vi "Operating Voltage.vi"(8 "error in (no error)":errorcluster) -> (0 "error out":errorcluster)   [LabVIEW 2025]
uses:
  SubVIs/All test cluster.ctl
  SubVIs/All_enum_ctl.ctl
  SubVIs/Arduino_lamps.ctl
  SubVIs/Lamps_global.vi
  <vilib>/Utility/file.llb/Write Delimited Spreadsheet (string).vi
  <instrlib>/BK Precision 9200 Series/BK Precision 9200 Series.lvlib
  <instrlib>/Keithley 2260B/Keithley 2260B.lvlib
panel:
  in  "ESP COM PORT":refnum<visa-resource-name>
  out "Connected? 2":bool caption="Long Blank Button"
  out "Status":string
  in  "POWER SUPPLY":bool caption="Blank Button"
  out "Text name":string
  in  "PS COM PORT":refnum<visa-resource-name>
  in  "Start/Stop":bool caption="Slide Switch"
  in  "File Path:":path
  in  "FILENAME":string
  out "Table":string[][](table)
  out "Connected?":bool caption="Long Blank Button"
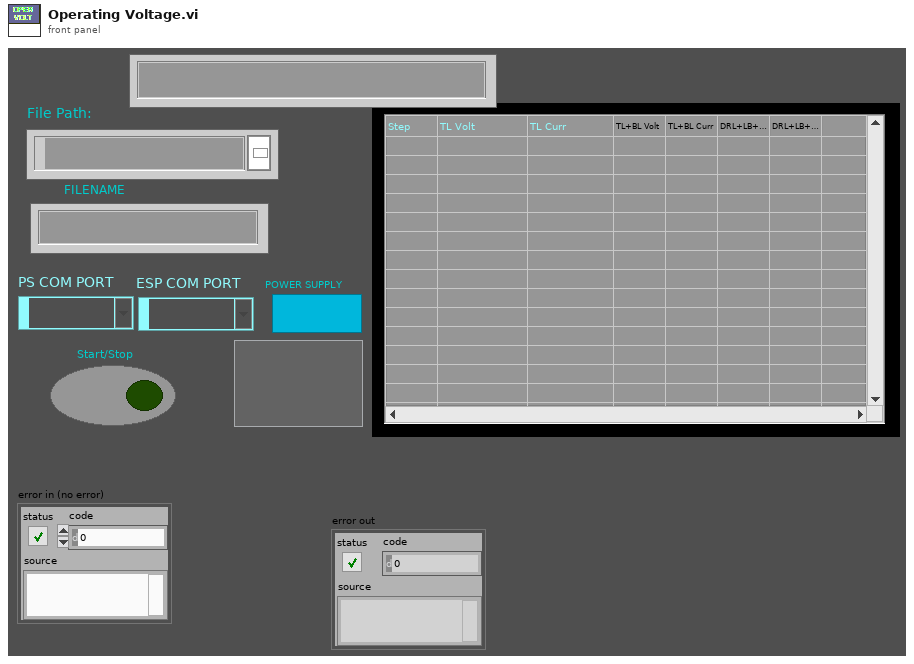
[diagram p1: front panel]
types:
  T1 = enum32{"Invalid", "Standard", "Closed", "Hidden", "Minimized", "Maximized"}
  T2 = typedef "All_enum_ctl.ctl" = enum16{"Init", "Poll", "Connect_esp32", "Connect", "check_start", "Start", "Set_Voltage", "On_relay", "Read_Voltage", "Off_Relay", "Next_Relay", "Next_Step", "Stop", "Store", "Error", "Exit"}
  T3 = typedef "All test cluster.ctl" = cluster{"FilePath":path, "Test Status":bool, "Start Volt":dbl, "End Volt":dbl, "Present Step":dbl, "Present Time(s)":dbl, "End Time":dbl, "Table":string[], "Intensity":string, "BK/Keith":bool, "COM":refnum<visa-resource-name>, "Next state":T2, "Step no.":dbl, "Start ms":u32, "ESP_COM":refnum<visa-resource-name>, "Relay_no":dbl, "Datas":string[]}
  T4 = typedef "Arduino_lamps.ctl" = enum16{"Init", "Poll", "Read", "Write", "Exit"}
  T5 = cluster{"Baud Rate":u32, "Parity":u16, "Data Bits":u16, "Stop Bits":u16, "Flow Control":u16}
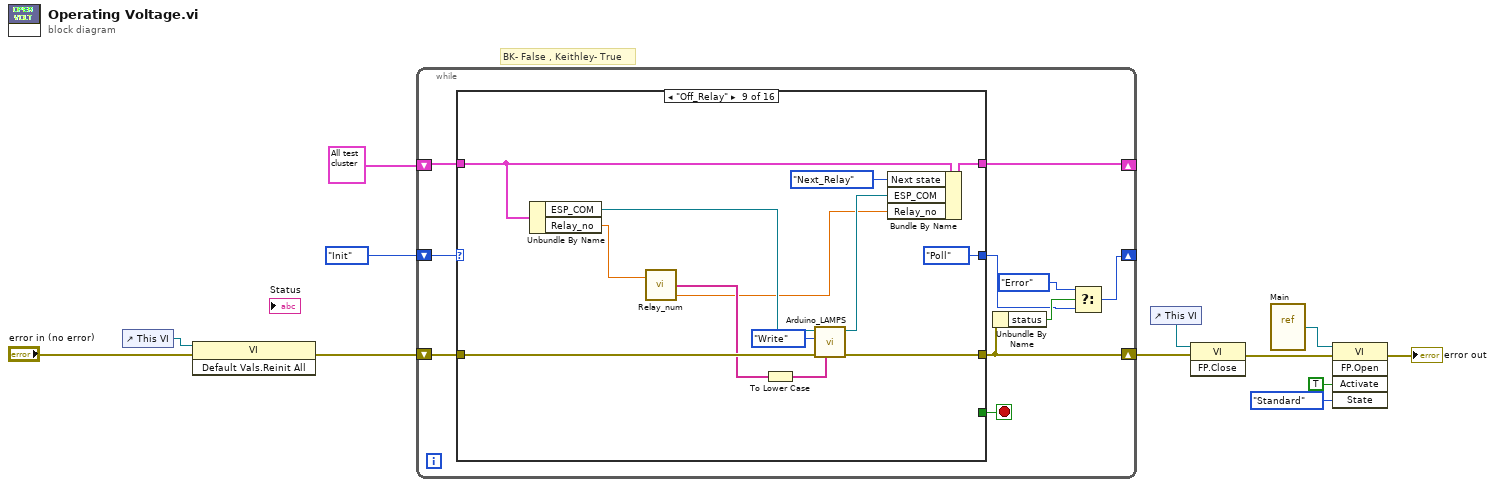
[diagram p0: block diagram]
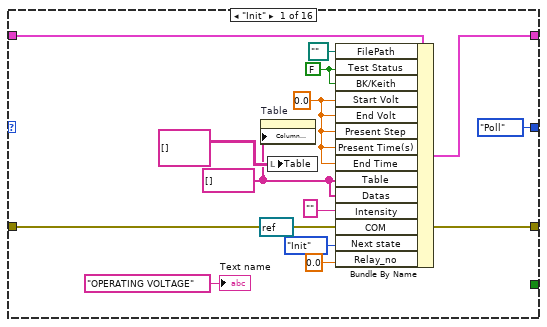
[diagram p2: hidden frame]
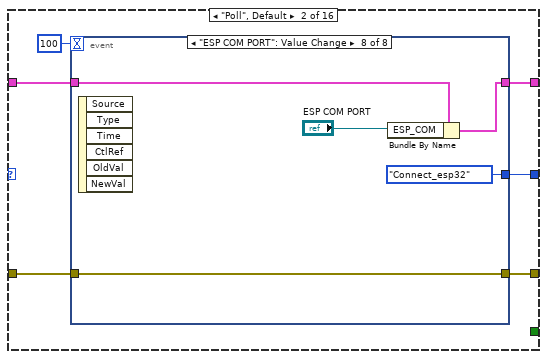
[diagram p3: hidden frame]
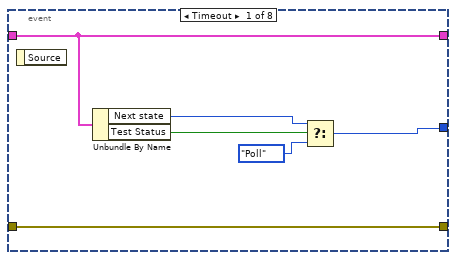
[diagram p4: hidden frame]
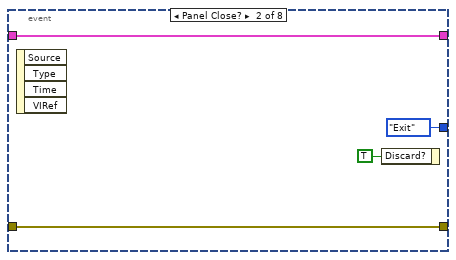
[diagram p5: hidden frame]
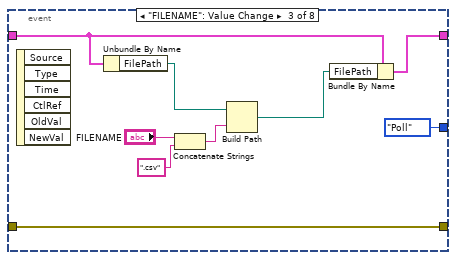
[diagram p6: hidden frame]
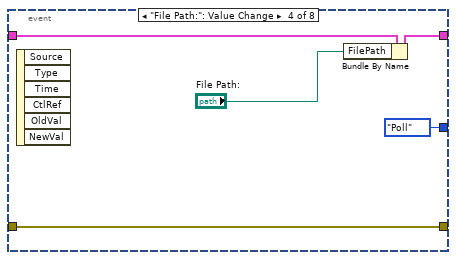
[diagram p7: hidden frame]
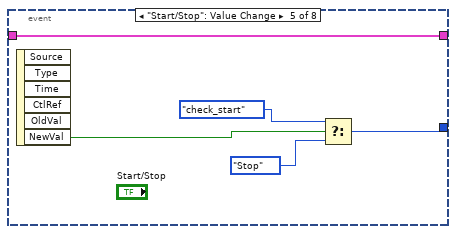
[diagram p8: hidden frame]
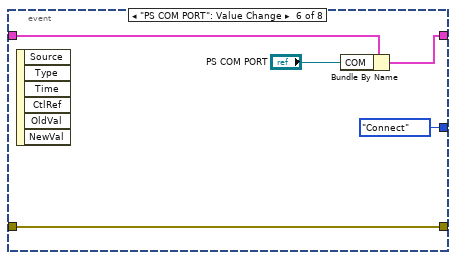
[diagram p9: hidden frame]
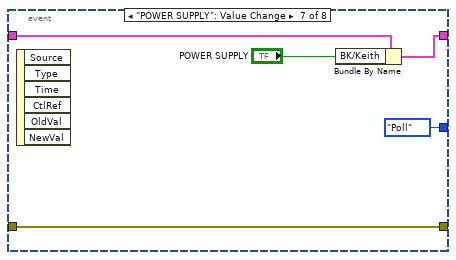
[diagram p10: hidden frame]
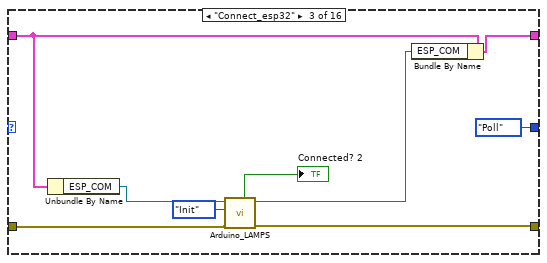
[diagram p11: hidden frame]
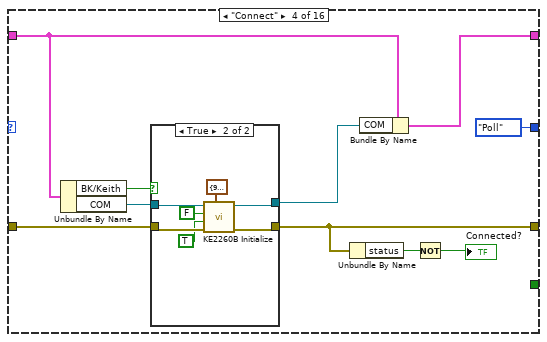
[diagram p12: hidden frame]
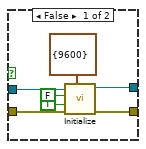
[diagram p13: hidden frame]
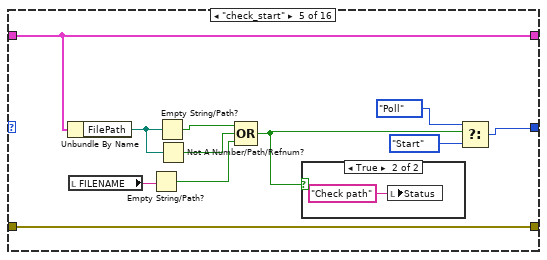
[diagram p14: hidden frame]
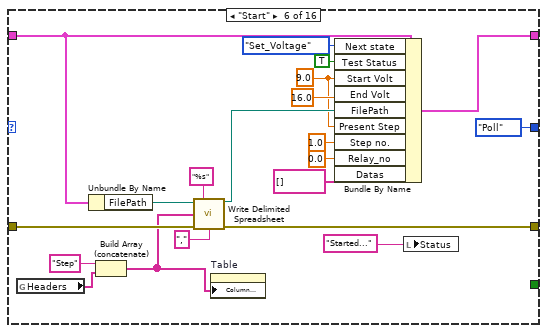
[diagram p16: hidden frame]
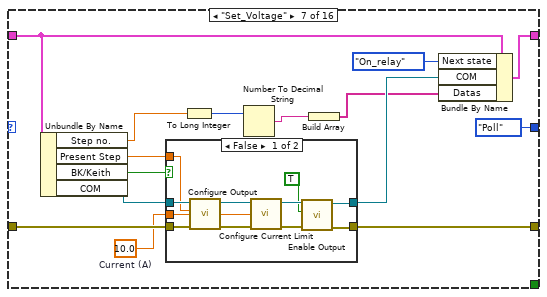
[diagram p17: hidden frame]
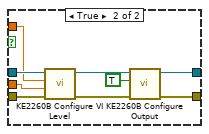
[diagram p18: hidden frame]
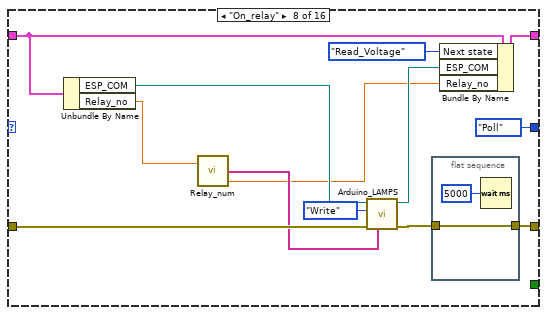
[diagram p19: hidden frame]
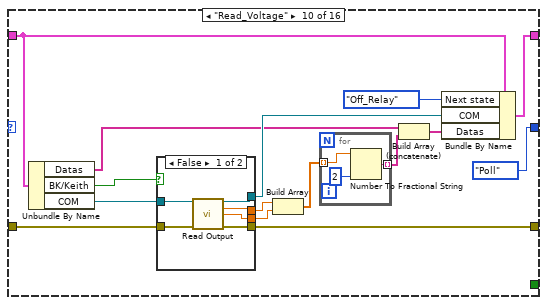
[diagram p20: hidden frame]
diagram:
  # "BK- False , Keithley- True"
  n1 = control-ref of="This VI"() -> (w12:refnum<vi>)
  n2 = invoke class="VI" method="Default Vals.Reinit All"(reference=w12, error in="error in (no error)") -> (error out=w10:errorcluster)  [unwired: 1 in, 2 out]
  n3 = while {
    shift-right: [w21] -> _
    shift-left: T3 {"FilePath"=path "", "Test Status"=FALSE, "Start Volt"=0.0, "End Volt"=0.0, "Present Step"=0.0, "Present Time(s)"=0.0, "End Time"=0.0, "Table"=[], "Intensity"="", "BK/Keith"=FALSE, "COM"="", "Next state"=enum."Init", "Step no."=0.0, "Start ms"=0, "ESP_COM"="", "Relay_no"=0.0, "Datas"=[]} -> [w20]
    shift-right: [w17] -> w2
    shift-left: w10 -> [w19]
    shift-right: [w13] -> _
    shift-left: All_enum_ctl."Init" -> [w22]
    stop <- w18 stop-if-true
    n4 = case shown="\"Off_Relay\"" w22 {
      tunnel: [w34 w39 w94 w97 w129 w150 w165 w194 w209 w224 w255 w265 w292 w306 w324 w344] -> w21
      tunnel: w20 -> [w36 w40 w93 w101 w129 w144 w164 w198 w213 w228 w258 w264 w290 w307 w327 w344]
      tunnel: w19 -> [w35 w42 w92 w105 w130 w146 w166 w199 w214 w229 w259 w267 w288 w311 w331 w349]
      tunnel: [w35 w41 w91 w100 w130 w145 w156 w190 w203 w227 w252 w267 w287 w311 w329 w345] -> w17
      tunnel: [All_enum_ctl."Poll" w37 All_enum_ctl."Poll" All_enum_ctl."Poll" w121 All_enum_ctl."Poll" All_enum_ctl."Poll" All_enum_ctl."Poll" All_enum_ctl."Poll" All_enum_ctl."Poll" All_enum_ctl."Poll" All_enum_ctl."Poll" All_enum_ctl."Poll" All_enum_ctl."Poll" All_enum_ctl."Poll" All_enum_ctl."Exit"] -> w14
      tunnel: [_ _ _ _ _ _ _ _ _ _ _ _ _ _ _ TRUE] -> w18
      frame "Init" {
        w23 = string[] [] ("Table")
        w32 = 0.0 ("Start Volt")
        w30 = FALSE ("Test Status")
        n5 = property on="Table" class="Tbl (strict)"("Column Headers[]"=w23) -> ()  [unwired: 2 in, 2 out]
        n6 = local write "Table"(string[][] [] ("Table")) -> ()
        n7 = Bundle By Name(cluster=w36, "FilePath"=path "", "Test Status"=w30, "BK/Keith"=w30, "Start Volt"=w32, "End Volt"=w32, "Present Step"=w32, "Present Time(s)"=w32, "End Time"=w32, "Table"=w23, "Datas"=w23, "Intensity"="", "COM"=refnum<visa-resource-name> refnum, "Next state"=All_enum_ctl."Init" ("Last state"), "Relay_no"=0.0) -> (w34:T3)
        "Text name" <- "OPERATING VOLTAGE" ("Text name")
      }
      frame "Poll", Default {
        n8 = event shown="[7] \"ESP COM PORT\": Value Change" {
          selector: _ -> [_ _ _ _ _ _ _ _]
          dyn-events: _ -> [_ _ _ _ _ _ _ _]
          timeout: 100 -> [_ _ _ _ _ _ _ _]
          tunnel: w42 -> [w48 w49 w61 w64 _ w72 w77 w82]
          tunnel: [w48 w49 w61 w64 _ w72 w77 w82] -> w41
          tunnel: w40 -> [w47 w50 w59 w66 w70 w76 w81 w85]
          tunnel: [w47 w50 w55 w63 w70 w75 w80 w86] -> w39
          tunnel: [w43 All_enum_ctl."Exit" ("f") All_enum_ctl."Poll" All_enum_ctl."Poll" w67 All_enum_ctl."Connect" ("f") All_enum_ctl."Poll" ("f") All_enum_ctl."Connect_esp32" ("f")] -> w37
          event Timeout {
            n9 = event-data() -> ()  [unwired: 1 in, 1 out]
            n10 = Unbundle By Name(w47) -> ("Next state"=w44:T2, "Test Status"=w46:bool)
            n11 = Select(t=w44, s=w46, f=All_enum_ctl."Poll") -> (s? t:f=w43:T2)
          }
          event Panel Close? {
            n12 = event-data() -> ()  [unwired: 1 in, 4 out]
            n13 = event-data("Discard?"=TRUE) -> ()  [unwired: 1 in, 1 out]
          }
          event "FILENAME": Value Change {
            n14 = event-data() -> ()  [unwired: 1 in, 6 out]
            n15 = Unbundle By Name(w59) -> ("FilePath"=w58:path)
            n16 = Concatenate Strings("FILENAME", ".csv" ("string")) -> (w57:string)
            n17 = Build Path(base path=w58, name or relative path=w57) -> (appended path=w54:path)
            n18 = Bundle By Name(cluster=w59, "FilePath"=w54) -> (w55:T3)
          }
          event "File Path:": Value Change {
            n19 = event-data() -> ()  [unwired: 1 in, 6 out]
            n20 = Bundle By Name(cluster=w66, "FilePath"="File Path:") -> (w63:T3)
          }
          event "Start/Stop": Value Change {
            n21 = event-data() -> ("NewVal"=w71:bool)  [unwired: 1 in, 5 out]
            n22 = Select(t=All_enum_ctl."check_start", s=w71, f=All_enum_ctl."Stop") -> (s? t:f=w67:T2)
          }
          event "PS COM PORT": Value Change {
            n23 = event-data() -> ()  [unwired: 1 in, 6 out]
            n24 = Bundle By Name(cluster=w76, "COM"="PS COM PORT") -> (w75:T3)
          }
          event "POWER SUPPLY": Value Change {
            n25 = event-data() -> ()  [unwired: 1 in, 6 out]
            n26 = Bundle By Name(cluster=w81, "BK/Keith"="POWER SUPPLY") -> (w80:T3)
          }
          event "ESP COM PORT": Value Change {
            n27 = event-data() -> ()  [unwired: 1 in, 6 out]
            n28 = Bundle By Name(cluster=w85, "ESP_COM"="ESP COM PORT") -> (w86:T3)
          }
        }
      }
      frame "Connect_esp32" {
        n29 = Unbundle By Name(w93) -> ("ESP_COM"=w89:refnum<visa-resource-name>)
        n30 = call "Arduino_LAMPS.vi"("error out"=w92, "Enum"=Arduino_lamps."Init", "VISA resource name"=w89) -> ("error out 2"=w91:errorcluster, "VISA out"=w88:refnum<visa-resource-name>, "status"=→"Connected? 2":bool)  [unwired: 4 in, 2 out]
        n31 = Bundle By Name(cluster=w93, "ESP_COM"=w88) -> (w94:T3)
      }
      frame "Connect" {
        n32 = Unbundle By Name(w101) -> ("BK/Keith"=w99:bool, "COM"=w98:refnum<visa-resource-name>)
        n33 = case shown="True" w99 {
          tunnel: w105 -> [w112 w119]
          tunnel: [w111 w118] -> w100
          tunnel: w98 -> [w110 w117]
          tunnel: [w106 w115] -> w96
          frame False {
            n34 = call <instrlib>:"Initialize.vi"("Serial Configuration"=cluster{"Baud Rate":u32} {"Baud Rate"=9600}, "error in (no error)"=w112, "Reset (True)"=TRUE, "ID Query (True)"=FALSE, "VISA resource name"=w110) -> ("error out"=w111:errorcluster, "VISA resource name out"=w106:refnum<visa-resource-name>)  [unwired: 5 in]
          }
          frame True {
            n35 = call <instrlib>:"KE2260B Initialize.vi"("Serial Configuration"=T5 {"Baud Rate"=9600, "Parity"=0, "Data Bits"=8, "Stop Bits"=10, "Flow Control"=0}, "error in (no error)"=w119, "Reset (True)"=TRUE, "ID Query (True)"=FALSE, "VISA resource name"=w117) -> ("error out"=w118:errorcluster, "VISA resource name out"=w115:refnum<visa-resource-name>)  [unwired: 5 in]
          }
        }
        n36 = Unbundle By Name(w100) -> ("status"=w104:bool)
        n37 = Bundle By Name(cluster=w101, "COM"=w96) -> (w97:T3)
        n38 = Not(x=w104) -> (.not. x?=→"Connected?":bool)
      }
      frame "check_start" {
        n39 = Unbundle By Name(w129) -> ("FilePath"=w127:path)
        n40 = local read "FILENAME"() -> (w128:string)
        n41 = Empty String/Path?(string/path=w128) -> (empty?=w124:bool)
        n42 = Empty String/Path?(string/path=w127) -> (empty?=w126:bool)
        n43 = Not A Number/Path/Refnum?(number/path/refnum=w127) -> (NaN/Path/Refnum?=w125:bool)
        n44 = Compound Arithmetic op=OR(w126, w125, w124) -> (w120:bool)
        n45 = case shown="True" w120 {
          frame False {
          }
          frame True {
            n46 = local write "Status"("Check path") -> ()
          }
        }
        n47 = Select(t=All_enum_ctl."Poll", s=w120, f=All_enum_ctl."Start") -> (s? t:f=w121:T2)
      }
      frame "Start" {
        w139 = 9.0 ("Start Volt")
        n48 = global read "Lamps_global.vi" "Headers"() -> (w133:string[])
        n49 = Unbundle By Name(w144) -> ("FilePath"=w143:path)
        n50 = Build Array (concatenate)("Step" ("String"), w133) -> (w132:string[])
        n51 = call-poly <vilib>:"Write Delimited Spreadsheet.vi"("file path (dialog if empty)"=w143, "format (%s)"="%s" ("format (%.3f)"), "1D data"=w132, "error in (no error)"=w146, "delimiter (\\t)"="," ("delimiter (\\t)")) -> ("new file path (Not A Path if cancelled)"=w140:path, "error out"=w145:errorcluster)  [unwired: 9 in]
        n52 = property on="Table" class="Tbl (strict)"("Column Headers[]"=w132) -> ()  [unwired: 2 in, 2 out]
        n53 = Bundle By Name(cluster=w144, "Next state"=All_enum_ctl."Set_Voltage" ("Last state"), "Test Status"=TRUE, "Start Volt"=w139, "End Volt"=16.0, "FilePath"=w140, "Present Step"=w139, "Step no."=1.0, "Relay_no"=0.0, "Datas"=string[] []) -> (w150:T3)
        n54 = local write "Status"("Started...") -> ()
      }
      frame "Set_Voltage" {
        w158 = 10.0  # Current (A)
        n55 = Unbundle By Name(w164) -> ("Step no."=w155:dbl, "Present Step"=w159:dbl, "BK/Keith"=w160:bool, "COM"=w163:refnum<visa-resource-name>)
        n56 = case shown="False" w160 {
          tunnel: w166 -> [w170 w186]
          tunnel: [w177 w185] -> w156
          tunnel: w163 -> [w175 w183]
          tunnel: [w176 w181] -> w162
          tunnel: w159 -> [w174 w179]
          tunnel: w158 -> [w168 w178]
          frame False {
            n57 = call <instrlib>:"Configure Output.vi"("error in (no error)"=w170, "Voltage Level (0.0 V)"=w174, "VISA resource name"=w175) -> ("error out"=w171:errorcluster, "VISA resource name out"=w169:refnum<visa-resource-name>)  [unwired: 7 in]
            n58 = call <instrlib>:"Configure Current Limit.vi"("error in (no error)"=w171, "Current Limit (0.0 A)"=w168, "VISA resource name"=w169) -> ("error out"=w173:errorcluster, "VISA resource name out"=w172:refnum<visa-resource-name>)  [unwired: 7 in]
            n59 = call <instrlib>:"Enable Output.vi"("error in (no error)"=w173, "Enable Output (F: False)"=TRUE, "VISA resource name"=w172) -> ("error out"=w177:errorcluster, "VISA resource name out"=w176:refnum<visa-resource-name>)  [unwired: 7 in]
          }
          frame True {
            n60 = call <instrlib>:"KE2260B Configure VI Level.vi"("error in (no error)"=w186, "Current Level (0.000 A)"=w178, "Voltage Level (0.000 V)"=w179, "VISA resource name"=w183) -> ("error out"=w184:errorcluster, "VISA resource name out"=w182:refnum<visa-resource-name>)  [unwired: 6 in]
            n61 = call <instrlib>:"KE2260B Configure Output.vi"("error in (no error)"=w184, "Enable Output (T: Enable)"=TRUE, "VISA resource name"=w182) -> ("error out"=w185:errorcluster, "VISA resource name out"=w181:refnum<visa-resource-name>)  [unwired: 7 in]
          }
        }
        n62 = To Long Integer(number=w155) -> (32bit integer=w154:i32)
        n63 = Number To Decimal String(number=w154) -> (decimal integer string=w153:string)  [unwired: 1 in]
        n64 = Build Array(w153) -> (w152:string[])
        n65 = Bundle By Name(cluster=w164, "Next state"=All_enum_ctl."On_relay", "COM"=w162, "Datas"=w152) -> (w165:T3)
      }
      frame "On_relay" {
        n66 = Unbundle By Name(w198) -> ("ESP_COM"=w197:refnum<visa-resource-name>, "Relay_no"=w189:dbl)
        n67 = call "Relay_num.vi"("Relay_no."=w189) -> ("Relay"=w188:string[], "Relay_no.out"=w187:dbl)  [unwired: 1 in, 1 out]
        n68 = call "Arduino_LAMPS.vi"("DO's"=w188, "error out"=w199, "Enum"=Arduino_lamps."Write", "VISA resource name"=w197) -> ("error out 2"=w191:errorcluster, "VISA out"=w193:refnum<visa-resource-name>)  [unwired: 3 in, 3 out]
        n69 = flat-sequence {
          tunnel: w191 -> [w201]
          tunnel: [w201] -> w190
          frame #0 {
            n70 = Wait (ms)(milliseconds to wait=u32 5000) -> ()  [unwired: 1 out]
          }
        }
        n71 = Bundle By Name(cluster=w198, "Next state"=All_enum_ctl."Read_Voltage", "ESP_COM"=w193, "Relay_no"=w187) -> (w194:T3)
      }
      frame "Off_Relay" {
        n72 = Unbundle By Name(w213) -> ("ESP_COM"=w212:refnum<visa-resource-name>, "Relay_no"=w206:dbl)
        n73 = call "Relay_num.vi"("Relay_no."=w206) -> ("Relay"=w205:string[], "Relay_no.out"=w204:dbl)  [unwired: 1 in, 1 out]
        n74 = To Lower Case(string=w205) -> (all lower case string=w202:string[])
        n75 = call "Arduino_LAMPS.vi"("DO's"=w202, "error out"=w214, "Enum"=Arduino_lamps."Write", "VISA resource name"=w212) -> ("error out 2"=w203:errorcluster, "VISA out"=w208:refnum<visa-resource-name>)  [unwired: 3 in, 3 out]
        n76 = Bundle By Name(cluster=w213, "Next state"=All_enum_ctl."Next_Relay", "ESP_COM"=w208, "Relay_no"=w204) -> (w209:T3)
      }
      frame "Read_Voltage" {
        n77 = Unbundle By Name(w228) -> ("Datas"=w216:string[], "BK/Keith"=w225:bool, "COM"=w226:refnum<visa-resource-name>)
        n78 = case shown="False" w225 {
          tunnel: w229 -> [w238 w244]
          tunnel: [w237 w243] -> w227
          tunnel: w226 -> [w236 w241]
          tunnel: [w235 w242] -> w223
          tunnel: [w234 w240] -> w220
          tunnel: [w233 w239] -> w219
          frame False {
            n79 = call <instrlib>:"Read Output.vi"("VISA resource name"=w236, "error in (no error)"=w238) -> ("VISA resource name out"=w235:refnum<visa-resource-name>, "Actual Voltage Level (V)"=w234:dbl, "Actual Current Level (A)"=w233:dbl, "error out"=w237:errorcluster)  [unwired: 9 in, 1 out]
          }
          frame True {
            n80 = call <instrlib>:"KE2260B Read Output.vi"("error in (no error)"=w244, "VISA resource name"=w241) -> ("error out"=w243:errorcluster, "Actual Current Level (A)"=w239:dbl, "Actual Voltage Level (V)"=w240:dbl, "VISA resource name out"=w242:refnum<visa-resource-name>)  [unwired: 6 in]
          }
        }
        n81 = Build Array(w220, w219) -> (w218:dbl[])
        n82 = for {
          tunnel: w218 -> [w231] mode=indexing
          tunnel: [w230] -> w217 mode=indexing
          n83 = Number To Fractional String(number=w231, precision (6)=i16 2) -> (F-format string=w230:string)  [unwired: 2 in]
        }
        n84 = Build Array (concatenate)(w216, w217) -> (w215:string[])
        n85 = Bundle By Name(cluster=w228, "Next state"=All_enum_ctl."Off_Relay", "COM"=w223, "Datas"=w215) -> (w224:T3)
      }
      frame "Store" {
        n86 = Unbundle By Name(w258) -> ("Table"=w249:string[], "FilePath"=w251:path)
        n87 = local read "Table"() -> (w257:string[][])
        n88 = Build Array (concatenate)(w257, w249) -> (→"Table":string[][])
        n89 = call-poly <vilib>:"Write Delimited Spreadsheet.vi"("file path (dialog if empty)"=w251, "format (%s)"="%s", "1D data"=w249, "append to file? (new file:F)"=TRUE, "error in (no error)"=w259, "delimiter (\\t)"="," ("delimiter (\\t)")) -> ("new file path (Not A Path if cancelled)"=w248:path, "error out"=w252:errorcluster)  [unwired: 8 in]
        n90 = Bundle By Name(cluster=w258, "Next state"=All_enum_ctl."Next_Step", "FilePath"=w248, "Datas"=string[] []) -> (w255:T3)
      }
      frame "Next_Relay" {
        n91 = Unbundle By Name(w264) -> ("Relay_no"=w263:dbl, "Datas"=w260:string[])
        n92 = call "Relay_num.vi"("Relay_no."=w263) -> ("x = y?"=w262:bool, "Relay_no.out"=w261:dbl)  [unwired: 1 in, 1 out]
        n93 = case shown="True" w262 {
          tunnel: [w277 w282] -> w265
          tunnel: w264 -> [w276 w281]
          tunnel: w261 -> [w274 _]
          tunnel: w260 -> [w268 w278]
          frame False {
            n94 = local read "Table"() -> (w272:string[][])
            n95 = Increment(x=w274) -> (x+1=w273:dbl)
            n96 = Array Size(array=w272) -> (size(s)=w270:i32[])
            n97 = Index Array(array=w270) -> (element=w269:i32)  [unwired: 1 in]
            n98 = Bundle By Name(cluster=w276, "Next state"=All_enum_ctl."On_relay", "Relay_no"=w273, "Datas"=w268) -> (w277:T3)
            n99 = Replace Array Subset(array=w272, new element=w268, index (row)=w269) -> (w271:string[][])  [unwired: 1 in]
            n100 = local write "Table"(w271) -> ()
          }
          frame True {
            n101 = Bundle By Name(cluster=w281, "Next state"=All_enum_ctl."Store", "Relay_no"=0.0, "Table"=w278) -> (w282:T3)
          }
        }
      }
      frame "Stop" {
        n102 = Unbundle By Name(w290) -> ("BK/Keith"=w285:bool, "COM"=w289:refnum<visa-resource-name>)
        n103 = case shown="False" w285 {
          tunnel: w288 -> [w296 w302]
          tunnel: [w298 w303] -> w287
          tunnel: w289 -> [w295 w301]
          tunnel: [w297 w300] -> w286
          frame False {
            n104 = call <instrlib>:"Enable Output.vi"("error in (no error)"=w296, "Enable Output (F: False)"=FALSE, "VISA resource name"=w295) -> ("error out"=w298:errorcluster, "VISA resource name out"=w297:refnum<visa-resource-name>)  [unwired: 7 in]
          }
          frame True {
            n105 = call <instrlib>:"KE2260B Configure Output.vi"("error in (no error)"=w302, "Enable Output (T: Enable)"=FALSE, "VISA resource name"=w301) -> ("error out"=w303:errorcluster, "VISA resource name out"=w300:refnum<visa-resource-name>)  [unwired: 7 in]
          }
        }
        n106 = local write "Start/Stop"(FALSE) -> ()
        n107 = Bundle By Name(cluster=w290, "Test Status"=FALSE, "COM"=w286) -> (w292:T3)
        n108 = local write "Status"("Test Stopped....") -> ()
      }
      frame "Next_Step" {
        n109 = Unbundle By Name(w307) -> ("Present Step"=w308:dbl, "End Volt"=w309:dbl, "Step no."=w304:dbl)
        n110 = Greater Or Equal?(x=w308, y=w309) -> (x >= y?=w310:bool)
        n111 = case shown="False" w310 {
          tunnel: w308 -> [w318 _]
          tunnel: w307 -> [w319 w322]
          tunnel: [w315 w321] -> w306
          tunnel: w304 -> [w313 _]
          frame False {
            n112 = Increment(x=w313) -> (x+1=w312:dbl)
            n113 = Add(x=w318, y=0.5) -> (x+y=w317:dbl)
            n114 = Bundle By Name(cluster=w319, "Next state"=All_enum_ctl."Set_Voltage", "Present Step"=w317, "Step no."=w312) -> (w315:T3)
          }
          frame True {
            n115 = Bundle By Name(cluster=w322, "Next state"=All_enum_ctl."Stop") -> (w321:T3)
          }
        }
      }
      frame "Error" {
        n116 = Unbundle By Name(w327) -> ("BK/Keith"=w325:bool, "COM"=w326:refnum<visa-resource-name>)
        n117 = case shown="False" w325 {
          tunnel: w331 -> [w334 w339]
          tunnel: [w335 w338] -> w328
          tunnel: w326 -> [w333 w337]
          tunnel: [w332 w336] -> w323
          frame False {
            n118 = call <instrlib>:"Reset.vi"("error in (no error)"=w334, "VISA resource name"=w333) -> ("error out"=w335:errorcluster, "VISA resource name out"=w332:refnum<visa-resource-name>)  [unwired: 8 in]
          }
          frame True {
            n119 = call <instrlib>:"KE2260B Reset.vi"("error in (no error)"=w339, "VISA resource name"=w337) -> ("error out"=w338:errorcluster, "VISA resource name out"=w336:refnum<visa-resource-name>)  [unwired: 8 in]
          }
        }
        n120 = call <vilib>:"Clear Errors.vi"("error in (no error)"=w328) -> ("error out"=w329:errorcluster)  [unwired: 5 in, 1 out]
        n121 = Bundle By Name(cluster=w327, "COM"=w323) -> (w324:T3)
      }
      frame "Exit" {
        n122 = Unbundle By Name(w344) -> ("ESP_COM"=w340:refnum<visa-resource-name>, "BK/Keith"=w342:bool, "COM"=w343:refnum<visa-resource-name>)
        n123 = case shown="False" w342 {
          tunnel: w349 -> [w352 w355]
          tunnel: [w351 w354] -> w346
          tunnel: w343 -> [w350 w353]
          frame False {
            n124 = call <instrlib>:"Close.vi"("error in (no error)"=w352, "VISA resource name"=w350) -> ("error out"=w351:errorcluster)  [unwired: 9 in]
          }
          frame True {
            n125 = call <instrlib>:"KE2260B Close.vi"("error in (no error)"=w355, "VISA resource name"=w353) -> ("error out"=w354:errorcluster)  [unwired: 9 in]
          }
        }
        n126 = VISA Close(VISA resource name=w340, error in (no error)=w346) -> (error out=w341:errorcluster)
        n127 = call <vilib>:"Clear Errors.vi"("error in (no error)"=w341) -> ("error out"=w345:errorcluster)  [unwired: 5 in, 1 out]
      }
    }
    n128 = Unbundle By Name(w17) -> ("status"=w16:bool)
    n129 = Select(t=All_enum_ctl."Error", s=w16, f=w14) -> (s? t:f=w13:T2)
  }
  n130 = control-ref of="This VI"() -> (w3:refnum<vi>)
  n131 = invoke class="VI" method="FP.Close"(reference=w3, error in=w2) -> (error out=w1:errorcluster)  [unwired: 1 in, 2 out]
  n132 = vi-ref "Main.vi"() -> (w7:refnum<vi>)
  n133 = invoke class="VI" method="FP.Open"(reference=w7, error in=w1, "Activate"=TRUE ("Activate?"), "State"=T1."Standard") -> (error out=→"error out":errorcluster)  [unwired: 1 in, 4 out]
